vi "getSerializedData.vi"(0 "reference":refnum<class "CallEdge.lvclass">, 5 "error in (no error)":errorcluster) -> (14 "reference out":refnum<class "CallEdge.lvclass">, 15 "startNode":refnum<class "AbstractNode.lvclass">, 16 "endNode":refnum<class "AbstractNode.lvclass">, 17 "xmlOut":string, 19 "error out":errorcluster)   [LabVIEW 2020, in "CallEdge.lvclass"]
doc: "getSerializedData"
uses:
  <resource>/Framework/Providers/Open_GDS/UML/CallEdge_class/CallEdge.lvclass
  C:/Program Files (x86)/National Instruments/LabVIEW 2020/resource/Framework/Providers/Open_GDS/UML/SegmentedLineEdge_class/SegmentedLineEdge.lvclass
  C:/Program Files (x86)/National Instruments/LabVIEW 2020/resource/Framework/Providers/Open_GDS/UML/AbstractEdge_class/AbstractEdge.lvclass
  <resource>/Framework/Providers/Open_GDS/UML/AbstractNode_class/AbstractNode.lvclass
  <resource>/Framework/Providers/Open_GDS/UML/General/Point/Point Point2D.ctl
  <resource>/Framework/Providers/Open_GDS/UML/ArrowHead_class/ArrowHead.lvclass
  <resource>/Framework/Providers/Open_GDS/UML/LineStyle_class/LineStyle.lvclass
  <resource>/Framework/Providers/Open_GDS/UML/SegmentedLineEdge_class/SegmentedLineEdge.lvclass
  <resource>/Framework/Providers/Open_GDS/UML/AbstractEdge_class/AbstractEdge.lvclass
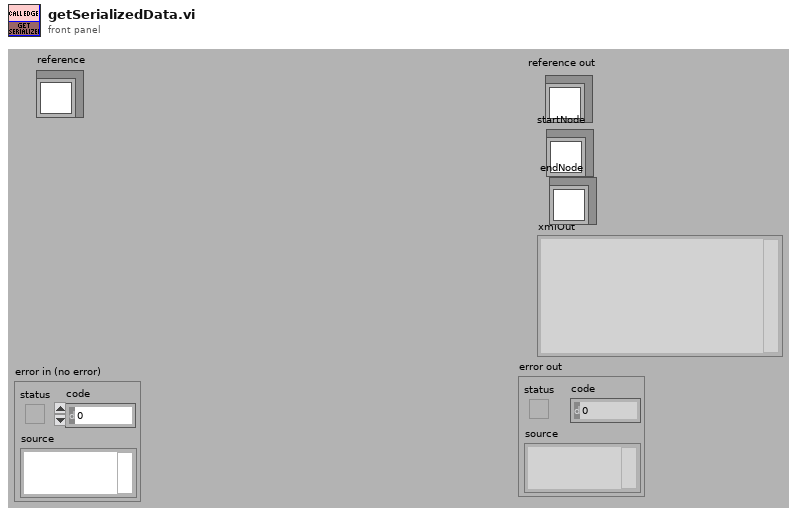
[diagram p1: front panel]
types:
  T1 = typedef "Point Point2D.ctl" = cluster{"x":dbl, "y":dbl}
  T2 = cluster{"Base class":cluster{"Base class":cluster{"Base class":cluster{"start":refnum<k1>, "end":refnum<k1>}}, "lineStyle":refnum<k1>, "startArrowHead":refnum<k1>, "endArrowHead":refnum<k1>, "startLabel":string, "midLabel":string, "endLabel":string, "MidLabelOffset":T1, "SplitWire":bool}, "signal":bool}
  T3 = typedef "CallEdge.lvclass/ObjectAttributes.ctl" = cluster{"signal":bool}
  T4 = typedef "SegmentedLineEdge.lvclass/ObjectAttributes.ctl" = cluster{"lineStyle":refnum<class "LineStyle.lvclass">, "startArrowHead":refnum<class "ArrowHead.lvclass">, "endArrowHead":refnum<class "ArrowHead.lvclass">, "startLabel":string, "midLabel":string, "endLabel":string, "MidLabelOffset":T1, "SplitWire":bool}
  T5 = typedef "AbstractEdge.lvclass/ObjectAttributes.ctl" = cluster{"start":refnum<class "AbstractNode.lvclass">, "end":refnum<class "AbstractNode.lvclass">}
  T6 = cluster{"Attributes":cluster{"Base class":cluster{"Base class":cluster{"Base class":cluster{"start":refnum<k1>, "end":refnum<k1>}}, "lineStyle":refnum<k1>, "startArrowHead":refnum<k1>, "endArrowHead":refnum<k1>, "startLabel":string, "midLabel":string, "endLabel":string, "MidLabelOffset":T1, "SplitWire":bool}, "signal":bool}, "Type(String)":string, "Object name":string, "Object name":string}
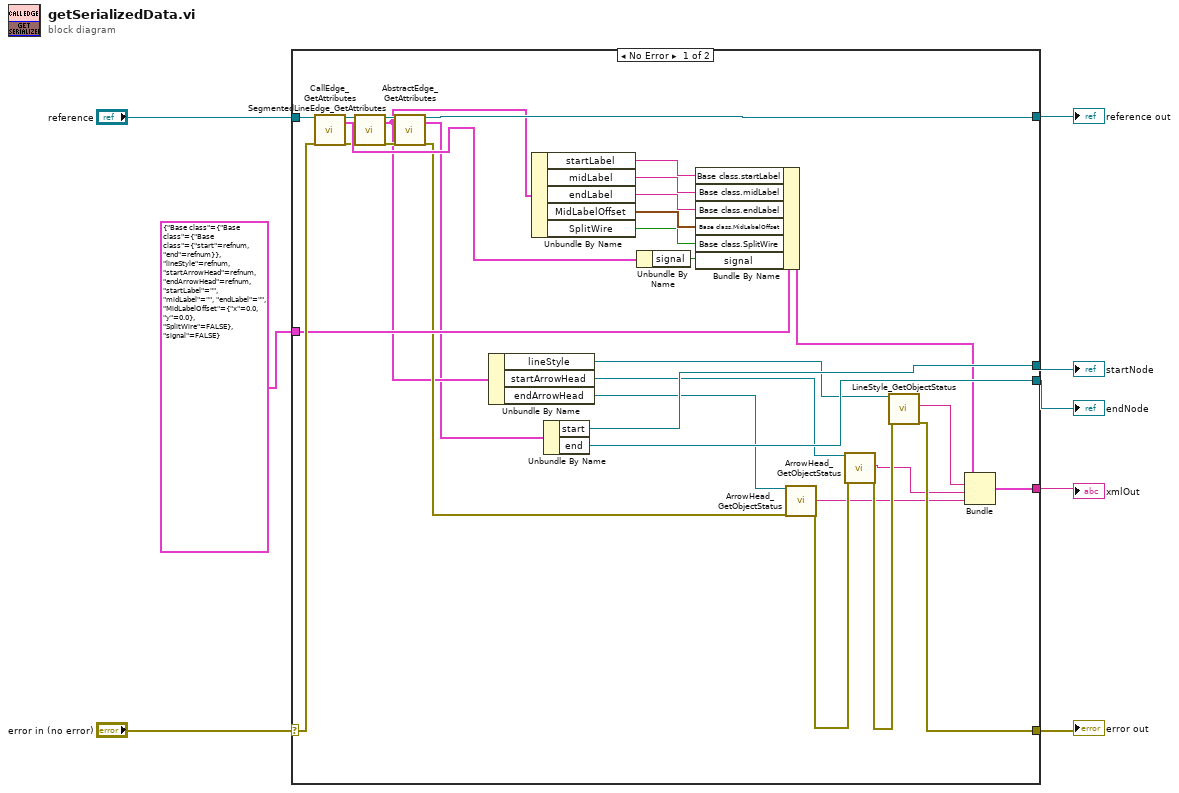
[diagram p0: block diagram]
diagram:
  n1 = case shown="No Error" "error in (no error)" {
    selector: "error in (no error)" -> [w40 w41]
    tunnel: "reference" -> [w39 w42]
    tunnel: [w29 w41] -> w6
    tunnel: [w14 w42] -> w5
    tunnel: [w37 _] -> w4
    tunnel: [w36 _] -> w3
    tunnel: [w35 _] -> w2
    tunnel: T2 {"Base class"={"Base class"={"Base class"={"start"=refnum, "end"=refnum}}, "lineStyle"=refnum, "startArrowHead"=refnum, "endArrowHead"=refnum, "startLabel"="", "midLabel"="", "endLabel"="", "MidLabelOffset"={"x"=0.0, "y"=0.0}, "SplitWire"=FALSE}, "signal"=FALSE} ("Attributes") -> [w28 _]
    frame No Error {
      n2 = call <resource>:"CallEdge_GetAttributes.vi"("reference in"=w39, "error in (no error)"=w40) -> ("reference out"=w19:refnum<class "CallEdge.lvclass">, "Data"=w20:T3, "error out"=w18:errorcluster)  [unwired: 1 in, 14 out]
      n3 = call <resource>:"SegmentedLineEdge_GetAttributes.vi"("reference in"=w19, "error in (no error)"=w18) -> ("reference out"=w17:refnum<class "CallEdge.lvclass">, "Data"=w13:T4, "error out"=w16:errorcluster)  [unwired: 14 in, 1 out]
      n4 = call <resource>:"AbstractEdge_GetAttributes.vi"("reference in"=w17, "error in (no error)"=w16) -> ("reference out"=w14:refnum<class "CallEdge.lvclass">, "Data"=w12:T5, "error out"=w15:errorcluster)  [unwired: 14 in, 1 out]
      n5 = Unbundle By Name(w13) -> ("lineStyle"=w34:refnum<class "LineStyle.lvclass">, "startArrowHead"=w33:refnum<class "ArrowHead.lvclass">, "endArrowHead"=w32:refnum<class "ArrowHead.lvclass">)
      n6 = Unbundle By Name(w13) -> ("startLabel"=w27:string, "midLabel"=w26:string, "endLabel"=w25:string, "MidLabelOffset"=w24:T1, "SplitWire"=w23:bool)
      n7 = Unbundle By Name(w12) -> ("start"=w36:refnum<class "AbstractNode.lvclass">, "end"=w35:refnum<class "AbstractNode.lvclass">)
      n8 = Unbundle By Name(w20) -> ("signal"=w22:bool)
      n9 = Bundle By Name(cluster=w28, "Base class.startLabel"=w27, "Base class.midLabel"=w26, "Base class.endLabel"=w25, "Base class.MidLabelOffset"=w24, "Base class.SplitWire"=w23, "signal"=w22) -> (w21:T2)
      n10 = call <resource>:"ArrowHead_GetObjectStatus.vi"("reference in"=w32, "error in (no error)"=w15) -> ("Object name"=w9:string, "error out"=w31:errorcluster)  [unwired: 1 in, 15 out]
      n11 = call <resource>:"ArrowHead_GetObjectStatus.vi"("reference in"=w33, "error in (no error)"=w31) -> ("Object name"=w10:string, "error out"=w30:errorcluster)  [unwired: 1 in, 15 out]
      n12 = call <resource>:"LineStyle_GetObjectStatus.vi"("reference"=w34, "error in (no error)"=w30) -> ("Type(String)"=w11:string, "error out"=w29:errorcluster)  [unwired: 15 in, 1 out]
      n13 = Bundle("Attributes"=w21, "Type(String)"=w11, "Object name"=w10, "Object name"=w9) -> (w38:T6)  [unwired: 1 out]
      n14 = Flatten To XML(6:w38) -> (2:w37:string)
    }
    frame Error {
    }
  }
  "reference out" <- w5
  "error out" <- w6
  "startNode" <- w3
  "endNode" <- w2
  "xmlOut" <- w4
